vi "Enqueue Return Value.vi"(8 "error in (no error)":errorcluster, 10 "Indicator Values":cluster{"Name":string, "Variant Data":variant}[](array[cluster]), 11 "Mock In":refnum<class "LMock Mock.lvclass">) -> (0 "error out":errorcluster, 3 "Mock Out":refnum<class "LMock Mock.lvclass">)   [LabVIEW 2020, in "LMock Mock.lvclass"]
uses:
  LMock Mock.lvclass
  LMock Mock.lvclass/LMock Mock.ctl
  Core/VI Call/VI Call.lvclass
  Parametric VI Call/Parametric VI Call.lvclass
  C:/git/astemes-lmock/source/Core/VI Call/VI Call.lvclass
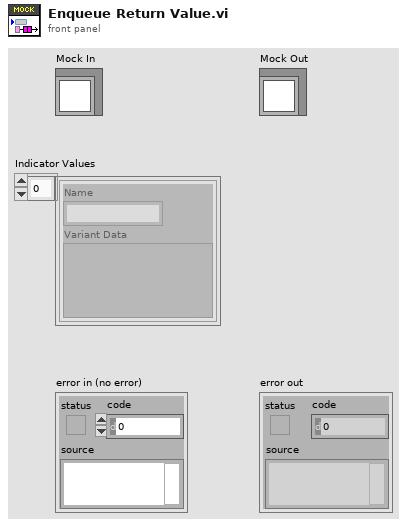
[diagram p1: front panel]
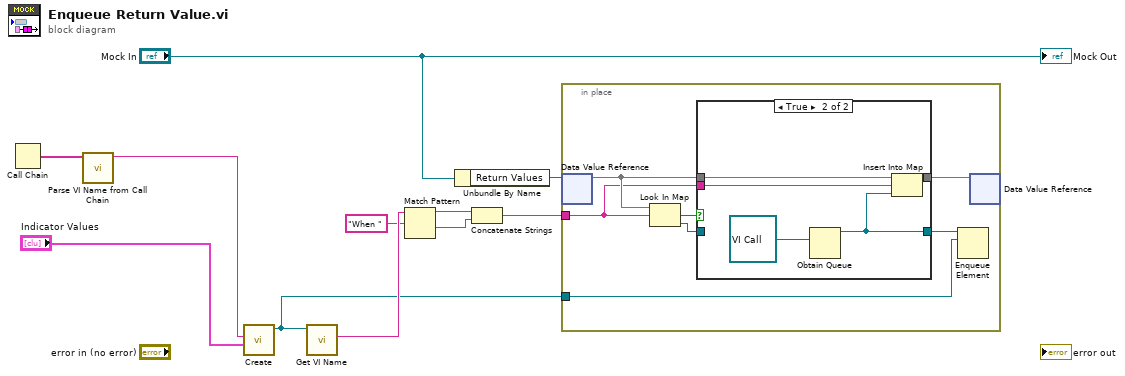
[diagram p0: block diagram]
diagram:
  n1 = Call Chain() -> (call chain=w2:string[])
  n2 = call "Parse VI Name from Call Chain.vi"("call chain"=w2) -> ("VI Name"=w1:string)  [unwired: 10 in]
  n3 = call "Create.vi"("Control Values"="Indicator Values", "VI Name"=w1) -> ("Parametric VI Call Out"=w4:refnum<class "Parametric VI Call.lvclass">)  [unwired: 9 in]
  n4 = call-dynamic "Get VI Name.vi"("Parametric VI Call In"=w4) -> ("VI Name"=w11:string)  [unwired: 10 in]
  n5 = Match Pattern(string=w11, regular expression="When ") -> (before substring=w9:string, after substring=w8:string)  [unwired: 1 in, 2 out]
  n6 = Unbundle By Name("Mock In") -> ("Return Values"=w6:refnum<data-value>)
  n7 = Concatenate Strings(w9, w8) -> (w5:string)
  n8 = in-place {
    in-place-border: w5 -> [w15]
    in-place-border: w4 -> [w12]
    n9 = in-place-dvr #1(w6) -> (w17:map{string, refnum<queue>})  [unwired: 1 out]
    n10 = Look In Map(map=w17, key=w15) -> (key not found?=w18:bool, value=w16:refnum<queue>)  [unwired: 1 in]
    n11 = case shown="True" w18 {
      tunnel: w17 -> [w20 w24]
      tunnel: w16 -> [w19 _]
      tunnel: w15 -> [_ w23]
      tunnel: [w20 w22] -> w14
      tunnel: [w19 w21] -> w13
      frame False {
      }
      frame True {
        n12 = Obtain Queue(element data type=refnum<class "VI Call.lvclass"> refnum ("Call Out")) -> (queue out=w21:refnum<queue>)  [unwired: 4 in, 2 out]
        n13 = Insert Into Map(map in=w24, key=w23, value=w21) -> (map out=w22:map{string, refnum<queue>})  [unwired: 2 out]
      }
    }
    n14 = Enqueue Element(queue=w13, element=w12) -> ()  [unwired: 2 in, 3 out]
    n15 = in-place-dvr #1(w14) -> ()  [unwired: 2 out]
  }
  "Mock Out" <- "Mock In"
